vi "FuncVI-FileGetDir.vi"(5 "InstanceRef":T2, 9 "arg list":T1[](array[typedef]) {"num" format="%.2f"}) -> (0 "error out":bool, 3 "result":T1 {"num" format="%.2f"})   [LabVIEW 2021]
doc: "::: CalcExpress Toolkit :::\nCopyright (c) 2000-2026 Konstantin Shifershteyn. All rights reserved."
uses:
  cetypes.llb/CalcExpress Function Argument Info.ctl
  cetypes.llb/CalcExpress Instance RefNum.ctl
panel:
  in  "max arg num":i32=1
  in  "min arg num":i32=1
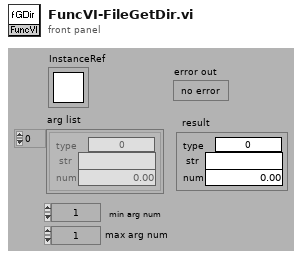
[diagram p1: front panel]
types:
  T1 = typedef "CalcExpress Function Argument Info.ctl" = cluster{"type":u32, "str":string, "num":dbl}
  T2 = typedef "CalcExpress Instance RefNum.ctl" = refnum<k1>
  T3 = enum32{"String", "DBL Number", "identifier", "1D Array of DBL", "2D Array of DBL", "CDB Number", "1D Array of CDB", "2D Array of CDB", "1D Array of String", "2D Array of String", "Unknown data type"}
  T4 = cluster{"type: use this constant to specify a predefined type code":enum32{"String", "DBL Number", "identifier", "1D Array of DBL", "2D Array of DBL", "CDB Number", "1D Array of CDB", "2D Array of CDB", "1D Array of String", "2D Array of String", "Unknown data type"}, string, dbl}
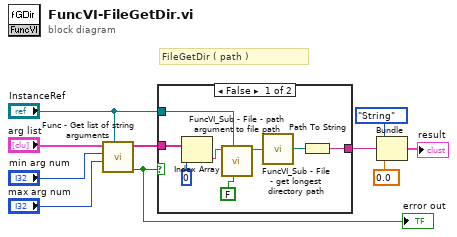
[diagram p0: block diagram]
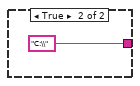
[diagram p2: hidden frame]
diagram:
  # "FileGetDir ( path )"
  n1 = call "Func - Get list of string arguments.vi"("InstanceRef"="InstanceRef", "max arg num"="max arg num", "min arg num"="min arg num", "arg list"="arg list") -> ("error out"=w3:bool, "val list"=w6:string[])  [unwired: 4 in]
  "error out" <- w3
  n2 = case shown="False" w3 {
    tunnel: "InstanceRef" -> [w15 _]
    tunnel: w6 -> [w16 _]
    tunnel: [w14 "C:\\"] -> w4
    frame False {
      n3 = Index Array(array=w16, index=0) -> (element=w17:string)
      n4 = call "FuncVI_Sub - File - path argument to file path.vi"("allow dialog"=FALSE, "InstanceRef"=w15, "arg: file path"=w17) -> ("file path"=w13:path)  [unwired: 6 in, 2 out]
      n5 = call "FuncVI_Sub - File - get longest directory path.vi"("path in"=w13) -> ("path out"=w12:path)  [unwired: 4 in]
      n6 = Path To String(path=w12) -> (string=w14:string)
    }
    frame True {
    }
  }
  n7 = Bundle("type: use this constant to specify a predefined type code"=T3."String", w4, 0.0) -> (→"result":T4)  [unwired: 1 in]
